vi "_CSM - Read File Logger Configuration - v1.0.vi"(5 "Section Name(\"FileLogger\")":string="FileLogger", 7 "error in (no error)":errorcluster) -> (1 "error out":errorcluster, 3 "FileLogger Configuration-v1":T1={"Enable"=TRUE, "Limit"={"FileSize"=10000000, "FileNum"=2}, "Timestamp.Format"="%<%Y/%m/%d %H:%M:%S%3u>T", "AutoExit"=FALSE} {"Limit"."FileSize" format="%.0p"})   [LabVIEW 2017, in "INI-Static-Variable-Support.lvlib"]
uses:
  INI-Static-Variable-Support.lvlib
  _fgv-oper.ctl
  <userlib>/_NEVSTOP/Communicable State Machine(CSM)/_Support/ChangeFlag/ChangeFlag-Read.vi
  <userlib>/_NEVSTOP/Communicable State Machine(CSM)/_Support/ChangeFlag/ChangeFlagDB.vi
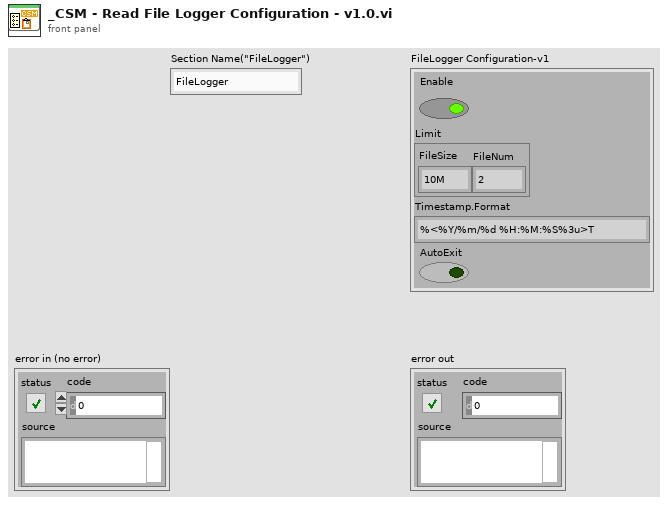
[diagram p1: front panel]
types:
  T1 = cluster{"Enable":bool, "Limit":cluster{"FileSize":i64, "FileNum":i32}, "Timestamp.Format":string, "AutoExit":bool}
  T2 = typedef "INI-Static-Variable-Support.lvlib/_fgv-oper.ctl" = enum16{"Read", "Write", "Sync", "Sessions", "List Keys", "Load", "List Files", "List Variables", "List Permanent Variables", "Mark Temp Variable as Permenent", "unload", "INIConfig(Memory)", "Reset", "Restore Variable Value"}
  T3 = typedef "LabVIEW-Config.lvlib/Config.ctl" = cluster{"Path":path, "Lines":string[], "Tokens":T4[], "Modified?":bool}
  T4 = typedef "LabVIEW-Config.lvlib/LineToken.ctl" = enum8{"comment", "section", "key", "more"}
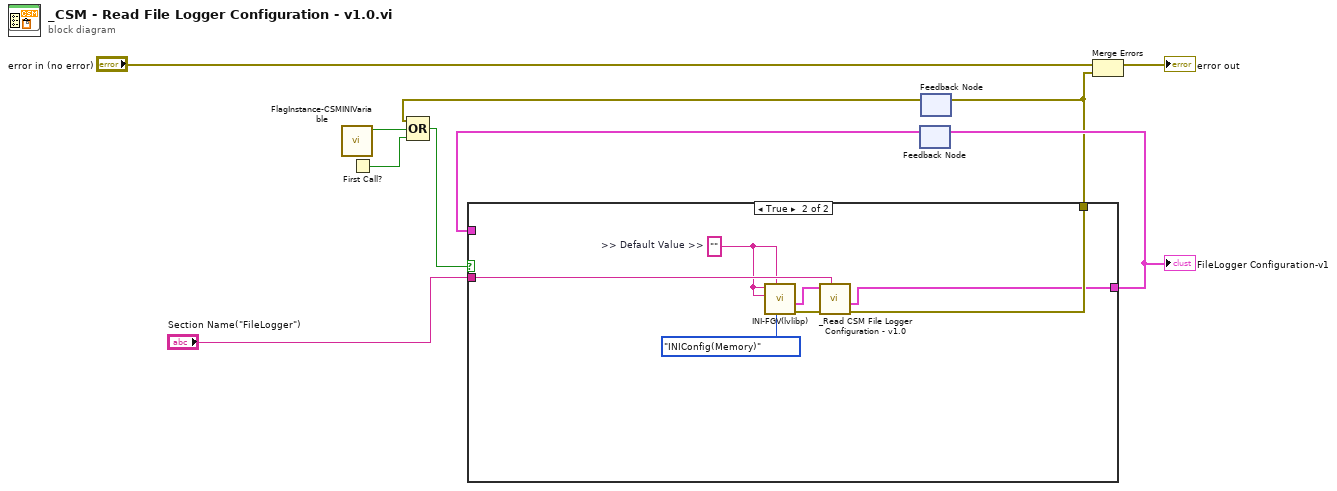
[diagram p0: block diagram]
diagram:
  n1 = call "FlagInstance-CSMINIVariable.vi"() -> ("Changed"=w1:bool)  [unwired: 10 in, 1 out]
  n2 = First Call?() -> (First Call?: T/F=w2:bool)
  n3 = feedback #1() -> (w7:T1)  [unwired: 1 in]
  n4 = feedback #2() -> (w5:errorcluster)  [unwired: 1 in]
  n5 = Compound Arithmetic op=OR(w5, w1, w2) -> (w4:bool)
  n6 = case shown="True" w4 {
    tunnel: [_ w16] -> w6
    tunnel: [w11 w15] -> w8
    tunnel: w7 -> [w11 _]
    tunnel: "Section Name(\"FileLogger\")" -> [_ w13]
    frame False {
    }
    frame True {
      w12 = ""  # >> Default Value >>
      n7 = call "INI-FGV(lvlibp).vi"("Enum"=_fgv-oper."INIConfig(Memory)", "Prefered Section"=w12, ">> Default Value >>"=w12, ">> Variable Name >>"=w12) -> ("error out"=w17:errorcluster, "INIConfig"=w14:T3)  [unwired: 4 in, 2 out]
      n8 = call "_Read CSM File Logger Configuration - v1.0.vi"("Section Name"=w13, "error in (no error)"=w17, "Config"=w14) -> ("error out"=w16:errorcluster, "FileLogger Configuration-v1"=w15:T1)  [unwired: 6 in, 1 out]
    }
  }
  "FileLogger Configuration-v1" <- w8
  n9 = feedback-in #1(w8) -> ()
  n10 = feedback-in #2(w6) -> ()
  n11 = Merge Errors("error in (no error)", w6) -> (→"error out":errorcluster)
